vi "demo1.vi"   [LabVIEW 2026]
uses:
  e88f81cd-5750-449a-a8d8-56df9929cb09.vi
  My Singleton Module.lvlib
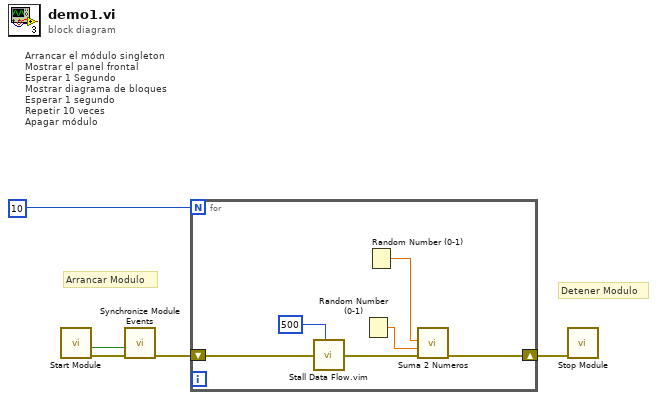
[diagram p0: block diagram]
diagram:
  # "Detener Modulo"
  # "Arrancar Modulo"
  # "Arrancar el módulo singleton\nMostrar el panel frontal\nEsperar 1 Segundo\nMostrar diagrama de bloques\nEsperar 1 segundo\nRepetir 10 veces\nApagar módulo"
  n1 = call "Start Module.vi"() -> ("error out"=w5:errorcluster, "Wait for Event Sync?"=w2:bool)  [unwired: 7 in, 3 out]
  n2 = call "Synchronize Module Events.vi"("error in"=w5, "Wait for Event Sync?"=w2) -> ("error out"=w4:errorcluster)  [unwired: 9 in]
  n3 = for {
    N: 10 -> [_]
    shift-right: [w8] -> w3
    shift-left: w4 -> [w11]
    n4 = call "Stall Data Flow.vim"("value in"=w11, "milliseconds to wait"=u32 500) -> ("value out"=w10:errorcluster)  [unwired: 1 out]
    n5 = Random Number (0-1)() -> (number: 0 to 1=w6:dbl)
    n6 = Random Number (0-1)() -> (number: 0 to 1=w7:dbl)
    n7 = call "Suma 2 Numeros.vi"("error in"=w10, "B"=w6, "A"=w7) -> ("error out"=w8:errorcluster)  [unwired: 6 in, 2 out]
  }
  n8 = call "Stop Module.vi"("error in"=w3) -> ()  [unwired: 10 in, 1 out]
